vi "Convert U64 Data to Image.vi"(7 "Image Data":u64[](array[numeric]), 8 "error in":errorcluster, 9 "Image Width":u32, 10 "Image Height":u32, 11 "Image Destination In":T1) -> (0 "error out":errorcluster, 3 "Image Destination Out":T1)   [LabVIEW 2013]
uses:
  <vilib>/vision/Image Controls.llb/IMAQ Image.ctl
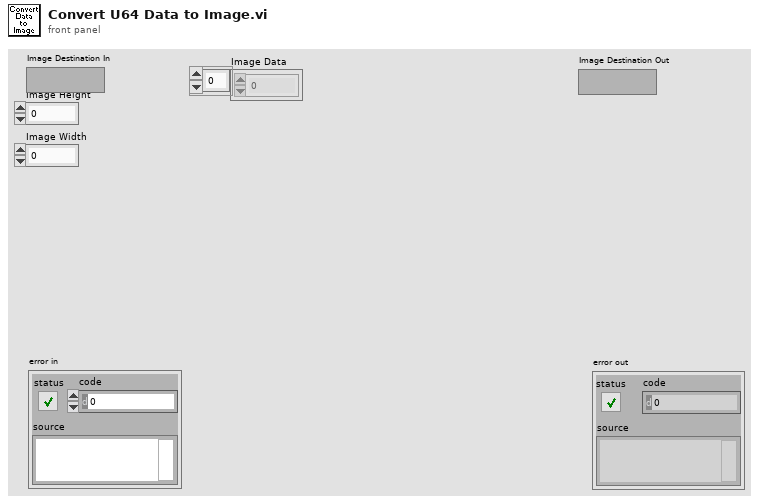
[diagram p1: front panel]
types:
  T1 = typedef "IMAQ Image.ctl" = refnum<image>
  T2 = enum16{"big-endian, network order", "native, host order", "little-endian"}
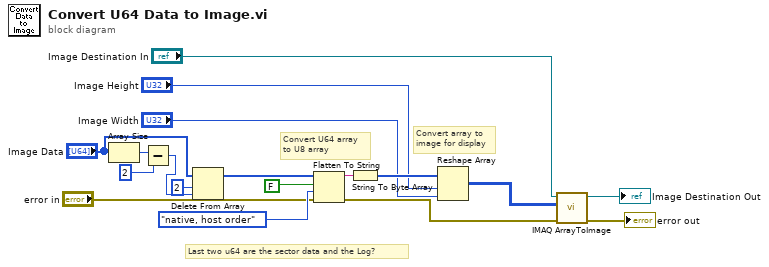
[diagram p0: block diagram]
diagram:
  # "Last two u64 are the sector data and the Log?"
  # "Convert U64 array\nto U8 array"
  # "Convert array to\nimage for display"
  n1 = Array Size(array="Image Data") -> (size(s)=w4:i32)
  n2 = Subtract(x=w4, y=2) -> (x-y=w1:i32)
  n3 = Delete From Array(array="Image Data", length=2, index=w1) -> (array with subset deleted=w6:u64[])  [unwired: 1 out]
  n4 = Flatten To String(anything=w6, prepend array or string size? (T)=FALSE, byte order (0:big-endian, network order)=T2."native, host order", error in (no error)="error in") -> (data string=w15:string, error out=w9:errorcluster)  [unwired: 1 out]
  n5 = String To Byte Array(string=w15) -> (unsigned byte array=w14:u8[])
  n6 = Reshape Array(w14, "Image Height", "Image Width") -> (w18:u8[][])
  n7 = call "IMAQ ArrayToImage"("error in (no error)"=w9, "Image Pixels (U8)"=w18, "Image"="Image Destination In") -> ("error out"=→"error out":errorcluster, "Image Out"=→"Image Destination Out":T1)  [unwired: 7 in]
